vi "Write VISA resource name.vi"(8 "error in (no error)":errorcluster, 10 "VISA resource name":refnum<visa-resource-name>, 11 "3D Controller in":refnum<class "3D Controller.lvclass">) -> (0 "error out":errorcluster, 3 "3D Controller out":refnum<class "3D Controller.lvclass">)   [LabVIEW 2023, in "FCC 3D Controller for BS.lvlib" / "3D Controller.lvclass"]
uses:
  3D Controller.lvclass
  3D Controller.lvclass/3D Controller.ctl
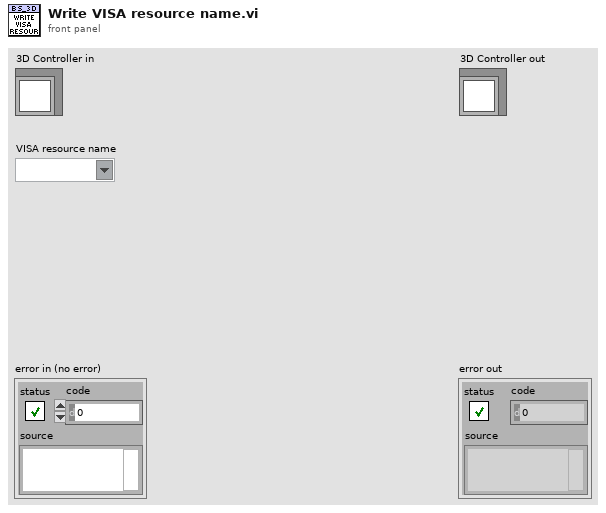
[diagram p1: front panel]
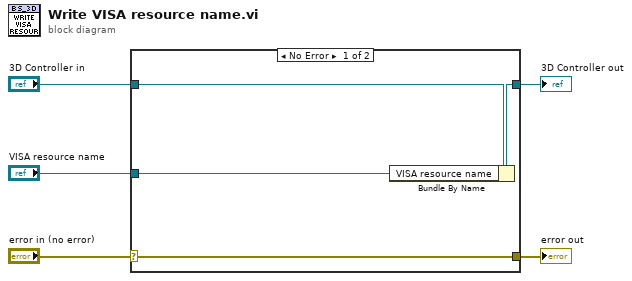
[diagram p0: block diagram]
diagram:
  n1 = case shown="No Error" "error in (no error)" {
    selector: "error in (no error)" -> [w9 w10]
    tunnel: [w9 w10] -> w4
    tunnel: [w7 w11] -> w2
    tunnel: "3D Controller in" -> [w8 w11]
    tunnel: "VISA resource name" -> [w6 _]
    frame No Error {
      n2 = Bundle By Name(cluster=w8, "VISA resource name"=w6) -> (w7:refnum<class "3D Controller.lvclass">)
    }
    frame Error {
    }
  }
  "error out" <- w4
  "3D Controller out" <- w2
